vi "PicoScope2000aExampleBlockAdvancedTrigger.vi"() -> ()   [LabVIEW 2010]
doc: "ps2000a API Block Capture example"
uses:
  shared/PicoBuffers.ctl
  <vilib>/Waveform/DWDTOps.llb/DWDT Analog to Digital.vi
  shared/Buffer and Transfer Settings.ctl
  shared/Acquisition Settings.ctl
  PicoScope2000aLib/PicoScope2000aAnalogChannelSettings.ctl
  PicoScope2000aLib/PicoScope2000aDigitalChannelSettings.ctl
panel:
  in  "Pulse Width Qualifier Settings":T1={"Direction"=2, "Lower Limit"=0, "Upper Limit"=0, "Pulse Width Type"=0} {"Pulse Width Type" items=["None", "Less Than", "Greater Than", "In Range", "Out of Range"]; "Direction" items=["Rising"=2, "Falling"=3]}
  in  "Pulse Width Qualifier Conditions":T2 {"Condition Logic" items=["AND", "OR", "XOR"]}
  in  "Auto Trigger (ms)":i32=1000
  in  "Channel A Trigger Properties":T3={"thresholdUpper"=0, "thresholdUpperHysteresis"=0, "thresholdLower"=0, "thresholdLowerHysteresis"=0, "Threshold Mode"=0, "Direction"=0, "Available"=TRUE} {"Direction" items=["Above / Inside", "Below / Outside", "Rising / Enter", "Falling / Exit", "Rising or Falling / Enter or Exit", "Above Lower", "Below Lower", "Rising Lower", "Falling Lower", "Positive Runt", "Negative Runt"]; "Threshold Mode" items=["Level", "Window"]}
  in  "Digital Port  0":T4 {"Direction Channel 7" items=["Don't Care", "Low", "High", "Rising", "Falling"]; "Direction Channel 6" items=["Don't Care", "Low", "High", "Rising", "Falling"]; "Direction Channel 5" items=["Don't Care", "Low", "High", "Rising", "Falling"]; "Direction Channel 4" items=["Don't Care", "Low", "High", "Rising", "Falling"]; "Direction Channel 3" items=["Don't Care", "Low", "High", "Rising", "Falling"]; "Direction Channel 2" items=["Don't Care", "Low", "High", "Rising", "Falling"]; "Direction Channel 1" items=["Don't Care", "Low", "High", "Rising", "Falling"]; "Direction Channel 0" items=["Don't Care", "Low", "High", "Rising", "Falling"]}
  in  "Trigger Conditions":T5 {"Condition Logic" items=["AND", "OR", "XOR"]}
  out "Properties Panel":T6 {"Max Total Capture Time Available (sec)" format="%.3p"; "Sample Frequency" format="%.3p"; "Sample Internal" format="%.3p"; "Max Samples Available" format="%.3p"; "Total Capture Time (sec)" format="%.3p"}
  in  "Port 0 Settings":T7={"Enabled"=FALSE, "Logic Level"=9830} {"Logic Level" items=["1.5V TTL"=9830, "2.5V CMOS"=16383]}
  in  "Channel A Settings":T8={"Enabled"=TRUE, "Coupling"=1, "Range"=6, "Analogue Offset"=0.0} {"Analogue Offset" format="%#_6p"; "Range" items=["20 mV"=1, "50 mV"=2, "100 mV"=3, "200 mV"=4, "500 mV"=5, "1 V"=6, "2 V"=7, "5 V"=8, "10 V"=9, "20 V"=10]; "Coupling" items=["AC", "DC"]}
  out "Device Info":T9={"Driver Version"="2.1.104.3324", "USB Version"="2.0", "Hardware"="1", "Variant"="2206A", "Batch and Serial"="CV676/049", "Cal Date"="19Sep17", "Kernel Version"="1.0", "Digital HW Version"="1", "Analogue HW Version"="1", "Firmware 1"="1.3.3.0", "Firmware 2"="0.5.47.0", "MSO"=FALSE, "Number of Channels"=2}
  out "overflow":i16 format="%06b"
  in  "Apply Settings":bool
  out "error out":errorcluster
  in  "Data file":path=path "PicoScope2000aExampleAdvancedTrgger ChA Data"
  in  "Buffer and Transfer Settings":T10={"startIndex"=0, "Samples"=32000, "Down Sample Ratio"=1, "Down-Sample Mode"=0} {"Down-Sample Mode" items=["RAW none"=2147483648, "None"=0, "Aggregate"=1, "Decimate"=2, "Average"=4]; "Down Sample Ratio" step=1; "Samples" format="%_6p"}
  in  "Acquisition Settings":T11={"preTriggerSamples"=0, "postTriggerSamples"=32000, "timebase"=5} {"postTriggerSamples" format="%_6p"; "preTriggerSamples" format="%_6p"}
  out "Port 0":digitalwaveform(graph)={"t0"=timestamp(0 s since 1904-01-01), "dt"=8e-09, "Y"={"transitions"=[], "data"=[]}}
  in  "stop":bool
  out "Analog Channels":cluster{i32, sgl, "Data":dbl[]}[](graph)
  in  "Serial Number":string
  in  "Use Serial Number":bool
  in  "error in (no error)":errorcluster
  # "Bit 0 = ChA"
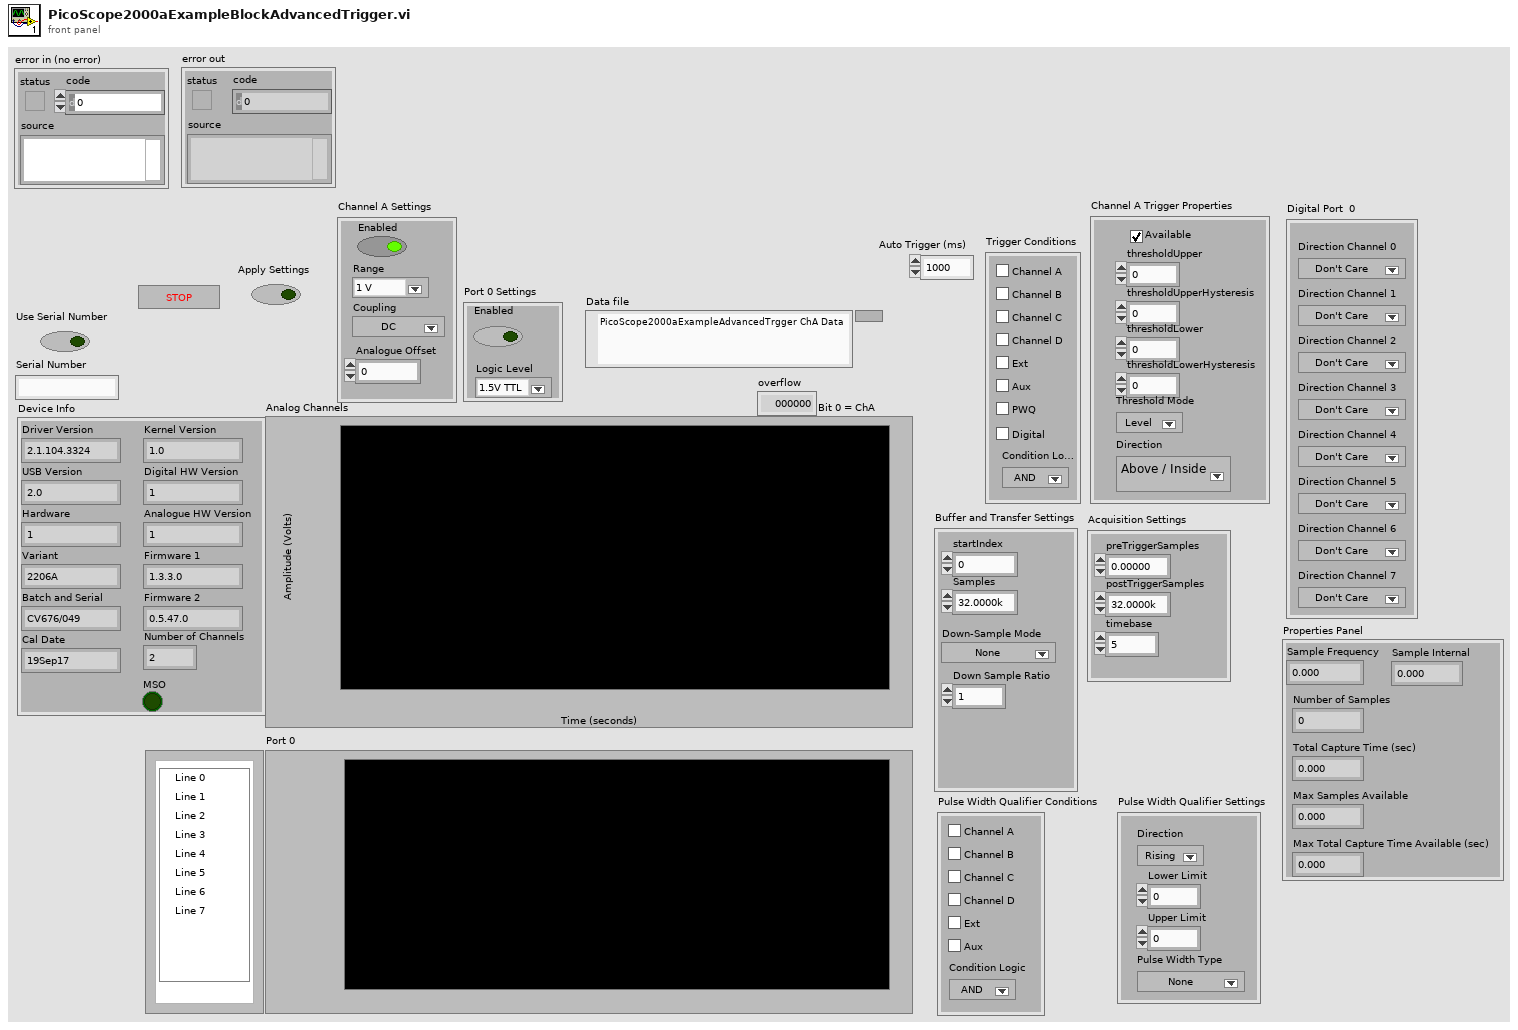
[diagram p1: front panel]
types:
  T1 = cluster{"Direction":i32, "Lower Limit":u32, "Upper Limit":u32, "Pulse Width Type":i32}
  T2 = cluster{"Channel A":bool, "Channel B":bool, "Channel C":bool, "Channel D":bool, "Aux":bool, "Condition Logic":u16, "Ext":bool}
  T3 = cluster{"thresholdUpper":i16, "thresholdUpperHysteresis":u16, "thresholdLower":i16, "thresholdLowerHysteresis":u16, "Threshold Mode":i32, "Direction":i32, "Available":bool}
  T4 = cluster{"Direction Channel 0":u16, "Direction Channel 1":u16, "Direction Channel 2":u16, "Direction Channel 3":u16, "Direction Channel 4":u16, "Direction Channel 5":u16, "Direction Channel 6":u16, "Direction Channel 7":u16}
  T5 = cluster{"Channel A":bool, "Channel B":bool, "Channel C":bool, "Channel D":bool, "Aux":bool, "PWQ":bool, "Condition Logic":u16, "Ext":bool, "Digital":bool}
  T6 = cluster{"Sample Frequency":sgl, "Sample Internal":sgl, "Max Samples Available":i32, "Number of Samples":u32, "Total Capture Time (sec) ":sgl, "Max Total Capture Time Available (sec)":sgl}
  T7 = typedef "PicoScope2000aDigitalChannelSettings.ctl" = cluster{"Enabled":bool, "Logic Level":i16}
  T8 = typedef "PicoScope2000aAnalogChannelSettings.ctl" = cluster{"Enabled":bool, "Coupling":i16, "Range":u16, "Analogue Offset":sgl}
  T9 = cluster{"Driver Version":string, "USB Version":string, "Hardware":string, "Variant":string, "Batch and Serial":string, "Cal Date":string, "Kernel Version":string, "Digital HW Version":string, "Analogue HW Version":string, "Firmware 1":string, "Firmware 2":string, "MSO":bool, "Number of Channels":i16}
  T10 = typedef "Buffer and Transfer Settings.ctl" = cluster{"startIndex":u64, "Samples":u64, "Down Sample Ratio":u64, "Down-Sample Mode":u32}
  T11 = typedef "Acquisition Settings.ctl" = cluster{"preTriggerSamples":u64, "postTriggerSamples":u64, "timebase":u32}
  T12 = enum16{"open", "open or create", "create or replace", "create", "open (read-only)"}
  T13 = typedef "PicoBuffers.ctl" = cluster{"Max Buffer Pointers":u64[][][], "Min Buffer Pointers":u64[][][], "StreamingDataInfo":cluster{"Channel":u32, "Down-Sample Mode":u32, "PICO_DATA_TYPE":enum32{"PICO_INT8_T", "PICO_INT16_T", "PICO_INT32_T", "PICO_UINT32_T", "PICO_INT64_T", ""}, "Samples":i32, "bufferIndex":u64, "startIndex":i32, "overflow":i16}[][]}
  T14 = cluster{"Channel A Buffer":i16[], "Channel B Buffer":i16[], "Channel C Buffer":i16[], "Channel D Buffer":i16[], "Channel E Buffer":i16[], "Channel F Buffer":i16[], "Channel G Buffer":i16[], "Channel H Buffer":i16[], "Port 0 Buffer":i16[], "Port 1 Buffer":i16[]}[]
  T15 = cluster{"Channel A Buffer":i16[], "Channel B Buffer":i16[], "Channel C Buffer":i16[], "Channel D Buffer":i16[], "Channel E Buffer":i16[], "Channel F Buffer":i16[], "Channel G Buffer":i16[], "Channel H Buffer":i16[], "Port 0 Buffer":i16[], "Port 1 Buffer":i16[]}
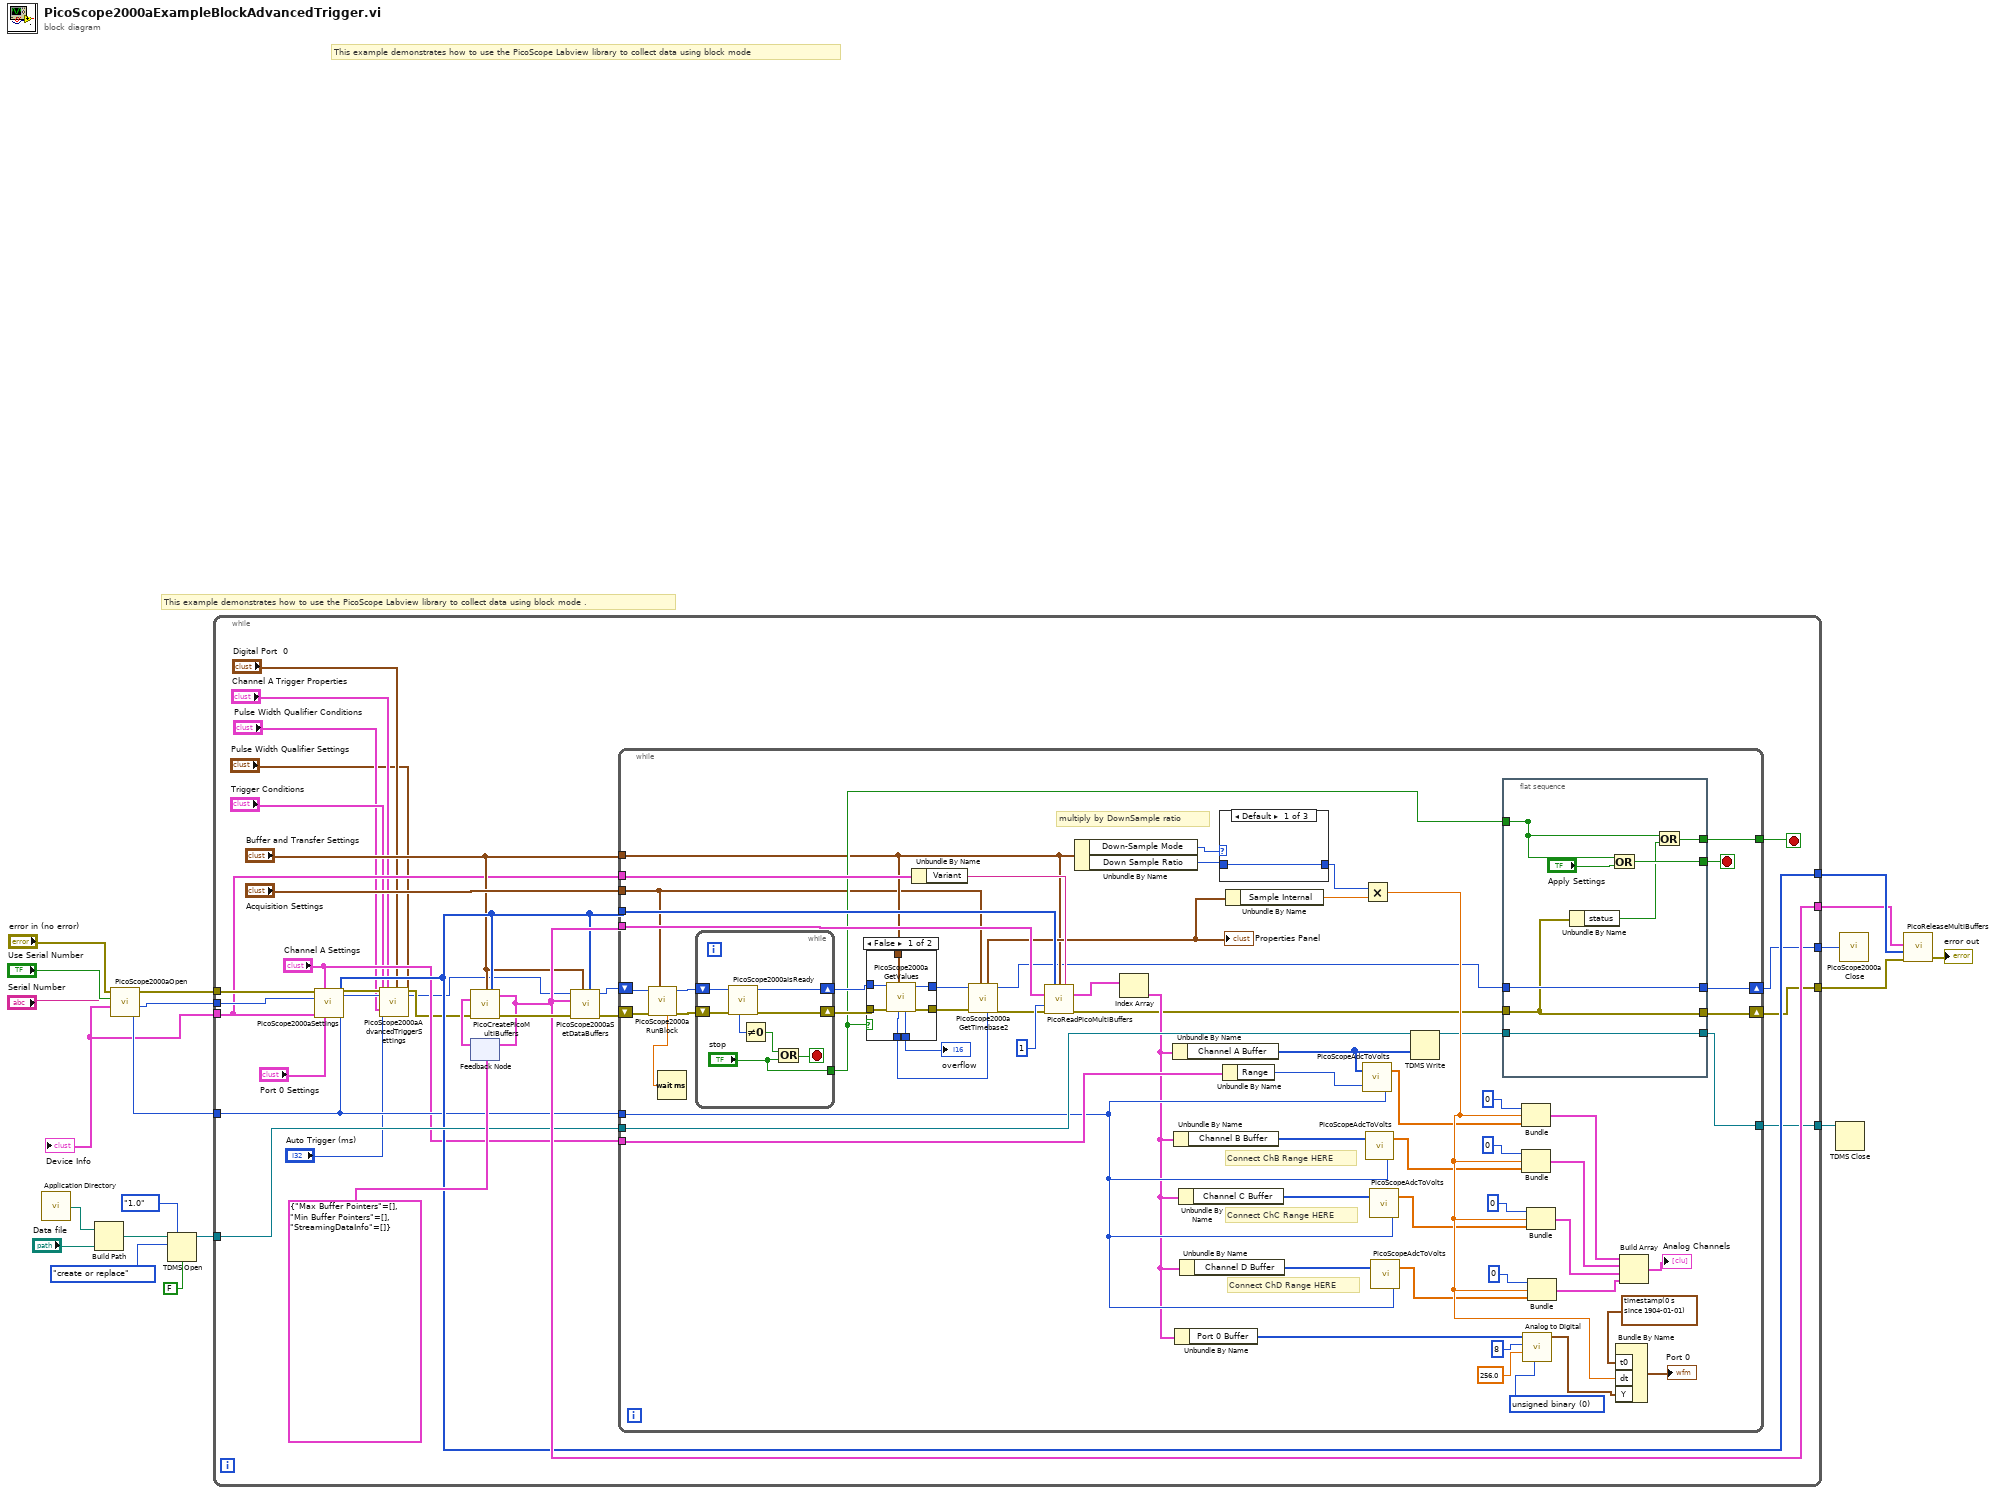
[diagram p0: block diagram]
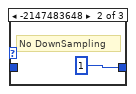
[diagram p3: hidden frame]
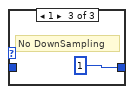
[diagram p4: hidden frame]
diagram:
  # "This example demonstrates how to use the PicoScope Labview library to collect data using block mode ."
  # "This example demonstrates how to use the PicoScope Labview library to collect data using block mode"
  n1 = call <vilib>:"Application Directory.vi"() -> ("Application Directory"=w12:path)
  n2 = Build Path(base path=w12, name or relative path="Data file") -> (appended path=w13:path)
  n3 = call "PicoScope2000aOpen.vi"("Serial Number"="Serial Number", "Use Serial Number"="Use Serial Number", "error in (no error)"="error in (no error)") -> ("Max Adc value"=w5:i16, "handle"=w20:i16, "error out"=w4:errorcluster, "Device Info"=w1:T9)  [unwired: 1 in]
  "Device Info" <- w1
  n4 = TDMS Open(6:FALSE ("disable buffering? (T)"), 7:enum16{"1.0", "2.0"}."1.0" ("file format version (2.0)"), 10:T12."create or replace" ("operation (0:open)"), 11:w13) -> (3:w10:refnum<k34>)  [unwired: 2 in, 1 out]
  n5 = while {
    tunnel: w20 -> [w45]
    tunnel: w5 -> [w41]
    tunnel: [w43] -> w19
    tunnel: [w47] -> w18
    tunnel: [w39] -> w11
    tunnel: w10 -> [w46]
    tunnel: w1 -> [w31]
    tunnel: w4 -> [w44]
    tunnel: [w40] -> w3
    tunnel: [w37] -> w2
    stop <- w38 stop-if-true
    n6 = call "PicoScope2000aSettings.vi"("error in"=w44, "Channel A Settings"="Channel A Settings", "handle in"=w45, "Port 0 Settings"="Port 0 Settings", "Device Info"=w31, "Max_adc"=w41) -> ("error out"=w30:errorcluster, "handle out"=w27:i16, "Enabled Array"=w43:i16[])  [unwired: 7 in]
    n7 = call "PicoScope2000aAdvancedTriggerSettings.vi"("error in"=w30, "handle in"=w27, "Trigger Conditions"="Trigger Conditions", "Auto Trigger (ms)"="Auto Trigger (ms)", "Channel A Trigger Properties"="Channel A Trigger Properties", "Digital Port  0"="Digital Port  0", "Pulse Width Qualifier Conditions"="Pulse Width Qualifier Conditions", "Pulse Width Qualifier Settings"="Pulse Width Qualifier Settings") -> ("error out"=w29:errorcluster, "handle out"=w28:i16)  [unwired: 10 in]
    n8 = feedback #1(T13 {"Max Buffer Pointers"=[], "Min Buffer Pointers"=[], "StreamingDataInfo"=[]} ("Data Pointers")) -> (w49:T13)
    n9 = call "PicoCreatePicoMultiBuffers.vi"("Buffer and Transfer Settings"="Buffer and Transfer Settings", "enabled array"=w43, "Data Pointers In"=w49, "error in (no error)"=w29) -> ("Data Pointers"=w47:T13, "error out"=w48:errorcluster)  [unwired: 10 in]
    n10 = feedback-in #1(w47) -> ()
    n11 = call "PicoScope2000aSetDataBuffers.vi"("enabled array"=w43, "Buffer and Transfer Settings"="Buffer and Transfer Settings", "error in (no error)"=w48, "Data Pointers In"=w47, "handle in"=w28) -> ("error out"=w36:errorcluster, "handle out"=w35:i16)  [unwired: 5 in]
    n12 = while {
      tunnel: w47 -> [w114]
      tunnel: "Buffer and Transfer Settings" -> [w56]
      tunnel: w43 -> [w105]
      tunnel: "Channel A Settings" -> [w104]
      tunnel: "Acquisition Settings" -> [w55]
      tunnel: w41 -> [w103]
      tunnel: w31 -> [w100]
      tunnel: [w68] -> w38
      shift-right: [w72] -> w40
      shift-left: w36 -> [w62]
      shift-right: [w66] -> w37
      shift-left: w35 -> [w63]
      tunnel: w46 -> [w113]
      tunnel: [w70] -> w39
      stop <- w67 stop-if-true
      w89 = u16 0 items=["unsigned binary", "offset binary", "2's complement"] ("data format (offset binary)")
      # "Connect ChB Range HERE"
      # "Connect ChD Range HERE"
      # "Connect ChC Range HERE"
      # "multiply by DownSample ratio"
      n13 = call "PicoScope2000aRunBlock.vi"("Acquisition Settings"=w55, "error in (no error)"=w62, "handle in"=w63) -> ("error out"=w107:errorcluster, "handle out"=w106:i16, "timeIndisposedMs"=w57:dbl)  [unwired: 5 in, 1 out]
      n14 = Wait (ms)(milliseconds to wait=w57) -> ()  [unwired: 1 out]
      n15 = while {
        shift-right: [w138] -> w64
        shift-left: w107 -> [w139]
        shift-right: [w137] -> w65
        shift-left: w106 -> [w136]
        tunnel: ["stop"] -> w61
        stop <- w133 stop-if-true
        n16 = call "PicoScope2000aIsReady.vi"("error in (no error)"=w139, "handle in"=w136) -> ("error out"=w138:errorcluster, "handle out"=w137:i16, "ready"=w135:i16)  [unwired: 7 in]
        n17 = Not Equal To 0?(x=w135) -> (x != 0?=w134:bool)
        n18 = Or(x=w134, y="stop") -> (x .or. y?=w133:bool)
      }
      n19 = case shown="False" w61 {
        tunnel: w64 -> [w121 w122]
        tunnel: w65 -> [w120 w123]
        tunnel: [w119 w123] -> w53
        tunnel: [w118 w122] -> w54
        tunnel: w56 -> [w117 _]
        tunnel: [w116 _] -> w60
        tunnel: [w115 _] -> w59
        frame False {
          n20 = call "PicoScope2000aGetValues.vi"("Buffer and Transfer Settings"=w117, "error in (no error)"=w121, "handle in"=w120) -> ("error out"=w118:errorcluster, "handle out"=w119:i16, "overflow"=w116:i16, "noOfSamples"=w115:u64)  [unwired: 5 in]
        }
        frame True {
        }
      }
      "overflow" <- w60
      n21 = Unbundle By Name(w100) -> ("Variant"=w101:string)
      n22 = call "PicoScope2000aGetTimebase2.vi"("Number of Samples"=w59, "Acquisition Settings"=w55, "error in (no error)"=w54, "handle in"=w53) -> ("error out"=w52:errorcluster, "handle out"=w51:i16, "Properties Panel"=w58:T6)  [unwired: 5 in]
      "Properties Panel" <- w58
      n23 = call "PicoReadPicoMultiBuffers.vi"("enabled array"=w105, "Buffer and Transfer Settings"=w56, "Variant"=w101, "Data Pointers"=w114, "No of Buffers"=1, "error in (no error)"=w52) -> ("MultiBuffers (Max or non-aggregated)"=w112:T14, "error out"=w69:errorcluster)  [unwired: 7 in, 1 out]
      n24 = Unbundle By Name(w56) -> ("Down-Sample Mode"=w110:u32, "Down Sample Ratio"=w111:u64)
      n25 = Index Array(array=w112) -> (element=w73:T15)  [unwired: 1 in]
      n26 = Unbundle By Name(w73) -> ("Channel A Buffer"=w82:i16[])
      n27 = Unbundle By Name(w73) -> ("Channel B Buffer"=w95:i16[])
      n28 = Unbundle By Name(w73) -> ("Port 0 Buffer"=w87:i16[])
      n29 = Unbundle By Name(w73) -> ("Channel C Buffer"=w80:i16[])
      n30 = Unbundle By Name(w73) -> ("Channel D Buffer"=w76:i16[])
      n31 = case shown="Default" w110 {
        tunnel: [w140 u64 1 ("Down Sample Ratio") u64 1 ("Down Sample Ratio")] -> w108
        tunnel: w111 -> [w140 _ _]
        frame Default {
        }
        frame -2147483648 {
          # "No DownSampling"
        }
        frame 1 {
          # "No DownSampling"
        }
      }
      n32 = Unbundle By Name(w104) -> ("Range"=w97:u16)
      n33 = Unbundle By Name(w58) -> ("Sample Internal"=w102:sgl)
      n34 = call "PicoScopeAdcToVolts.vi"("Max_adc"=w103, "Range Index"=w97, "Data"=w82) -> ("Data"=w83:dbl[])
      n35 = Multiply(x=w108, y=w102) -> (x*y=w109:sgl)
      n36 = call "PicoScopeAdcToVolts.vi"("Max_adc"=w103, "Data"=w95) -> ("Data"=w94:dbl[])  [unwired: 1 in]
      n37 = call "PicoScopeAdcToVolts.vi"("Max_adc"=w103, "Data"=w80) -> ("Data"=w79:dbl[])  [unwired: 1 in]
      n38 = call "PicoScopeAdcToVolts.vi"("Max_adc"=w103, "Data"=w76) -> ("Data"=w75:dbl[])  [unwired: 1 in]
      n39 = TDMS Write(0:w113, 9:w82) -> (4:w71:refnum<k34>)  [unwired: 4 in, 3 out]
      n40 = flat-sequence {
        tunnel: [w131] -> w67
        tunnel: [w124] -> _
        tunnel: [w128] -> w68
        tunnel: w51 -> [w127]
        tunnel: [w127] -> w66
        tunnel: w69 -> [w126]
        tunnel: [w126] -> w72
        tunnel: [w125] -> w70
        tunnel: w71 -> [w125]
        tunnel: w61 -> [w124]
        frame #0 {
          n41 = Unbundle By Name(w126) -> ("status"=w129:bool)
          n42 = Or(x=w124, y="Apply Settings") -> (x .or. y?=w131:bool)
          n43 = Or(x=w124, y=w129) -> (x .or. y?=w128:bool)
        }
      }
      n44 = Bundle(0, w109, "Data"=w83) -> (w93:cluster{i32, sgl, "Data":dbl[]})  [unwired: 1 in]
      n45 = Bundle(0, w109, "Data"=w94) -> (w92:cluster{i32, sgl, "Data":dbl[]})  [unwired: 1 in]
      n46 = call-poly <vilib>:"Analog to Digital.vi"("data format (offset binary)"=w89, "full-scale range (pk-pk)"=256.0, "resolution (16 bit)"=8, "analog waveform"=w87) -> ("digital waveform"=w84:digitalwaveform)  [unwired: 4 in, 3 out]
      n47 = Bundle(0, w109, "Data"=w79) -> (w78:cluster{i32, sgl, "Data":dbl[]})  [unwired: 1 in]
      n48 = Bundle(0, w109, "Data"=w75) -> (w74:cluster{i32, sgl, "Data":dbl[]})  [unwired: 1 in]
      n49 = Bundle By Name("t0"=timestamp(0 s since 1904-01-01), "dt"=w109, "Y"=w84) -> (→"Port 0":digitalwaveform)  [unwired: 1 in]
      n50 = Build Array(w93, w92, w78, w74) -> (→"Analog Channels":cluster{i32, sgl, "Data":dbl[]}[])
    }
  }
  n51 = TDMS Close(11:w11) -> ()  [unwired: 1 in, 2 out]
  n52 = call "PicoScope2000aClose.vi"("handle"=w2) -> ()
  n53 = call "PicoReleaseMultiBuffers.vi"("error in (no error)"=w3, "Enabled array"=w19, "Data Pointers"=w18) -> ("error out"=→"error out":errorcluster)  [unwired: 8 in]
